vi "onGenerateStreamEvent.vi"(6 "Session ID":i32, 8 "error in (no error)":errorcluster, 9 "Direction":T1, 10 "Bytes":u8[](array[numeric]) format="%02x", 11 "DebuggingTerminal in":refnum<class "DebuggingTerminal.lvclass">) -> (0 "error out":errorcluster, 3 "DebuggingTerminal out":refnum<class "DebuggingTerminal.lvclass">)   [LabVIEW 2013, in "MQTT Base.lvlib" / "DebuggingTerminal.lvclass"]
uses:
  DebuggingTerminal.lvclass
  Stream Direction -- enum.ctl
  Stream Data -- cluster.ctl
  DebuggingTerminal.lvclass/DebuggingTerminal.ctl
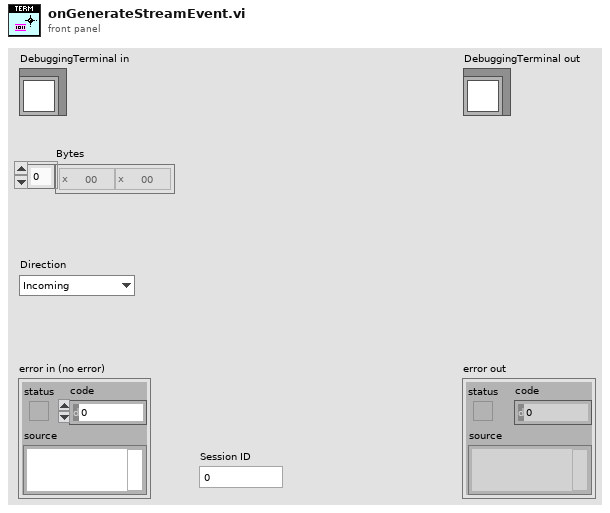
[diagram p1: front panel]
types:
  T1 = typedef "MQTT Base.lvlib/DebuggingTerminal.lvclass/Stream Direction -- enum.ctl" = enum16{"Incoming", "Outgoing"}
  T2 = typedef "MQTT Base.lvlib/DebuggingTerminal.lvclass/Stream Data -- cluster.ctl" = cluster{"Session ID":i32, "Bytes":u8[]}
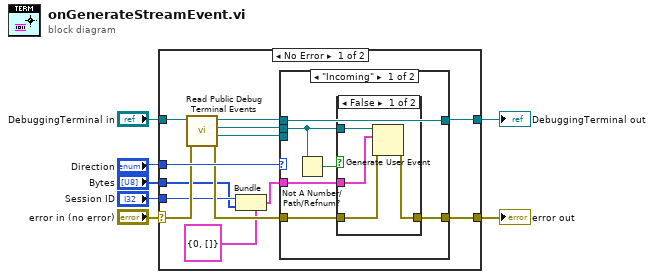
[diagram p0: block diagram]
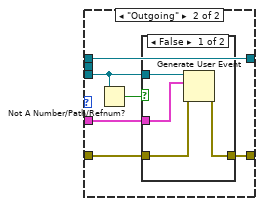
[diagram p3: hidden frame]
diagram:
  n1 = case shown="No Error" "error in (no error)" {
    selector: "error in (no error)" -> [w16 w44]
    tunnel: [w12 w44] -> w6
    tunnel: [w20 w43] -> w4
    tunnel: "DebuggingTerminal in" -> [w18 w43]
    tunnel: "Direction" -> [w19 _]
    tunnel: "Bytes" -> [w10 _]
    tunnel: "Session ID" -> [w11 _]
    frame No Error {
      n2 = call "Read Public Debug Terminal Events.vi"("error in (no error)"=w16, "DebuggingTerminal in"=w18) -> ("error out"=w13:errorcluster, "Outgoing Stream"=w14:refnum<user-event>, "Incoming Stream"=w15:refnum<user-event>, "DebuggingTerminal out"=w17:refnum<class "DebuggingTerminal.lvclass">)  [unwired: 6 in]
      n3 = Bundle(cluster=T2 {"Session ID"=0, "Bytes"=[]} ("stream"), "Session ID"=w11, "Bytes"=w10) -> (w9:T2)
      n4 = case shown="\"Incoming\"" w19 {
        tunnel: [w26 w37] -> w20
        tunnel: w17 -> [w26 w37]
        tunnel: w15 -> [w25 _]
        tunnel: w14 -> [_ w33]
        tunnel: w9 -> [w23 w36]
        tunnel: w13 -> [w22 w35]
        tunnel: [w21 w34] -> w12
        frame "Incoming" {
          n5 = Not A Number/Path/Refnum?(number/path/refnum=w25) -> (NaN/Path/Refnum?=w24:bool)
          n6 = case shown="False" w24 {
            tunnel: w23 -> [w30 _]
            tunnel: w22 -> [w29 w31]
            tunnel: [w28 w31] -> w21
            tunnel: w25 -> [w27 _]
            frame False {
              n7 = Generate User Event(user event=w27, event data cluster=w30, error in=w29) -> (error out=w28:errorcluster)  [unwired: 1 in, 1 out]
            }
            frame True {
            }
          }
        }
        frame "Outgoing" {
          n8 = Not A Number/Path/Refnum?(number/path/refnum=w33) -> (NaN/Path/Refnum?=w32:bool)
          n9 = case shown="False" w32 {
            tunnel: w36 -> [w41 _]
            tunnel: w35 -> [w40 w42]
            tunnel: [w39 w42] -> w34
            tunnel: w33 -> [w38 _]
            frame False {
              n10 = Generate User Event(user event=w38, event data cluster=w41, error in=w40) -> (error out=w39:errorcluster)  [unwired: 1 in, 1 out]
            }
            frame True {
            }
          }
        }
      }
    }
    frame Error {
    }
  }
  "error out" <- w6
  "DebuggingTerminal out" <- w4
